vi "VIH HelpGen - Write HTML File - VI - VI Description.vi"(4 "InstanceRef":string, 6 "Description Params":cluster{"DscrMode":T3, "Description":string}, 7 "Save params":T1, 8 "error in":errorcluster, 9 "Original VI Info":cluster{"VI Name":string, "Conpane Image":T2}, 10 "HTML in":string, 11 "VI Reference":refnum<vi>) -> (0 "error out":errorcluster, 2 "HTML out":string, 3 "dup VI Reference":refnum<vi>)   [LabVIEW 2014]
doc: "::: VI Helpeks :::\nCopyright (c) 2000-2026 Konstantin Shifershteyn. All rights reserved."
uses:
  VIH HelpGen Typedef - Enum - Description Mode.ctl
  <vilib>/picture/picture.llb/imagedata.ctl
panel:
  out "ALL FOUND":bool
  # "VI Helpeks\nCopyright (c) 2012-2026 Konstantin Shifershteyn"
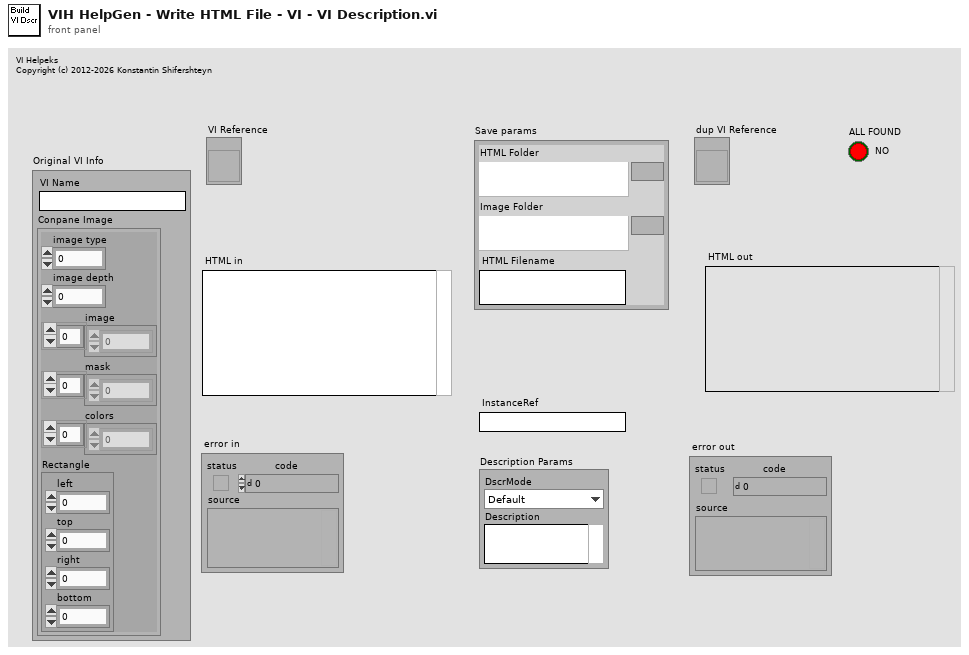
[diagram p1: front panel]
types:
  T1 = cluster{"HTML Folder":path, "Image Folder":path, "HTML Filename":string}
  T2 = typedef "imagedata.ctl" = cluster{"image type":i32, "image depth":i32, "image":u8[], "mask":u8[], "colors":u32[], "Rectangle":cluster{"left":i16, "top":i16, "right":i16, "bottom":i16}}
  T3 = typedef "VIH HelpGen Typedef - Enum - Description Mode.ctl" = enum16{"Default", "Description", "Description1", "Description2", "Custom", "None"}
  T4 = typedef "VIH HelpGen Typedef - Control Terminal Attributes Cluster.ctl" = cluster{"Conpane Idx":i32, "Control":bool, "Wire Rule":enum16{"Invalid Wire Rule", "Required", "Recommended", "Optional", "Dynamic Dispatch"}}
  T5 = cluster{"Ctrl ID":string, "Conpane Idx":i32, "Bounds":cluster{"X0":i32, "Y0":i32, "X1":i32, "Y1":i32}}[]
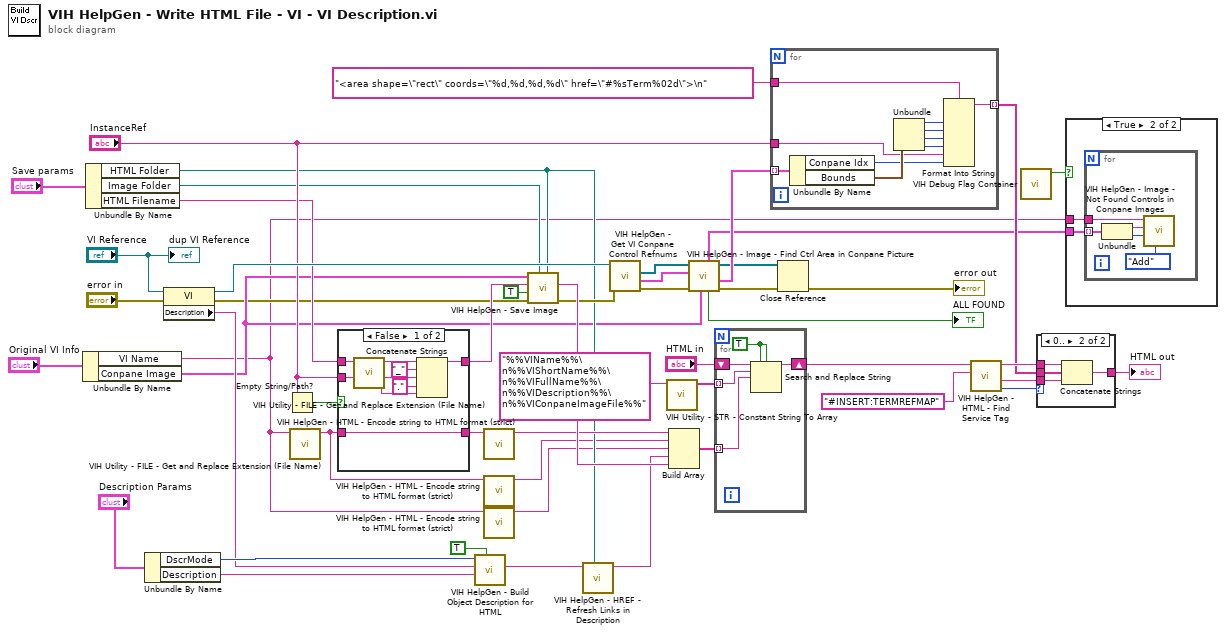
[diagram p0: block diagram]
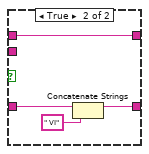
[diagram p3: hidden frame]
diagram:
  n1 = Unbundle By Name("Original VI Info") -> ("VI Name"=w4:string, "Conpane Image"=w6:T2)
  n2 = Unbundle By Name("Save params") -> ("HTML Folder"=w9:path, "Image Folder"=w8:path, "HTML Filename"=w7:string)
  n3 = Unbundle By Name("Description Params") -> ("DscrMode"=w27:T3, "Description"=w25:string)
  n4 = property class="VI"(reference="VI Reference", error in="error in") -> (reference out=w42:refnum<vi>, error out=w5:errorcluster, "Description"=w26:string)
  n5 = Empty String/Path?(string/path="InstanceRef") -> (empty?=w18:bool)
  n6 = call "VIH Utility - FILE - Get and Replace Extension (File Name).vi"("File name"=w4) -> ("File name out"=w3:string)  [unwired: 9 in, 1 out]
  n7 = case shown="False" w18 {
    tunnel: w3 -> [w59 w61]
    tunnel: [w59 w60] -> w14
    tunnel: [w58 w62] -> w11
    tunnel: w7 -> [w55 w62]
    tunnel: "InstanceRef" -> [w56 _]
    frame False {
      n8 = call "VIH Utility - FILE - Get and Replace Extension (File Name).vi"("File name"=w55) -> ("extension"=w53:string, "File name out"=w54:string)  [unwired: 9 in]
      n9 = Concatenate Strings(w54, "_" ("string"), w56, "." ("string"), w53) -> (w58:string)
    }
    frame True {
      n10 = Concatenate Strings(w61, " VI") -> (w60:string)
    }
  }
  n11 = call "VIH HelpGen - Build Object Description for HTML.vi"("Ena \"No Description\" message (F)"=TRUE ("Ena \"No Description\" message (F)"), "Custom Description"=w25, "Default Description"=w26, "DscrMode"=w27) -> ("Description HTML out"=w20:string)  [unwired: 6 in, 1 out]
  n12 = call "VIH HelpGen - HTML - Encode string to HTML format (strict).vi"("string"=w14) -> ("HTML string"=w13:string)  [unwired: 10 in]
  n13 = call "VIH HelpGen - HTML - Encode string to HTML format (strict).vi"("string"=w3) -> ("HTML string"=w2:string)  [unwired: 10 in]
  n14 = call "VIH HelpGen - HTML - Encode string to HTML format (strict).vi"("string"=w4) -> ("HTML string"=w1:string)  [unwired: 10 in]
  n15 = call "VIH HelpGen - Save Image.vi"("HTML Folder"=w9, "Image Folder"=w8, "error in"=w5, "Always overwrite (F)"=TRUE, "Image Filename"=w11, "image data"=w6) -> ("error out"=w43:errorcluster, "path for HTML"=w45:string)  [unwired: 3 in, 1 out]
  n16 = call "VIH HelpGen - HREF - Refresh Links in Description.vi"("HTML Folder"=w9, "Description in"=w20) -> ("Description out"=w19:string)  [unwired: 9 in]
  n17 = call "VIH HelpGen - Get VI Conpane Control Refnums.vi"("error in"=w43, "VI Reference"=w42) -> ("error out"=w41:errorcluster, "Ctrl Attributes"=w21:T4[], "Conpane Ctrl Refnums"=w23:refnum<vi>[])  [unwired: 6 in, 1 out]
  n18 = call "VIH Utility - STR - Constant String To Array.vi"("String in"="%%VIName%%\n%%VIShortName%%\n%%VIFullName%%\n%%VIDescription%%\n%%VIConpaneImageFile%%") -> ("Array out"=w49:string[])  [unwired: 10 in]
  n19 = Build Array(w13, w2, w1, w19, w45) -> (w48:string[])
  n20 = call "VIH HelpGen - Image - Find Ctrl Area in Conpane Picture.vi"("Conpane Image Data"=w6, "error in"=w41, "Ctrl Attributes"=w21, "Conpane Ctrl Refnums"=w23) -> ("error out"=w40:errorcluster, "Terminals Info"=w33:T5, "dup Conpane Ctrl Refnums"=w22:refnum<vi>[], "ALL FOUND"=→"ALL FOUND":bool, "Not Found"=w16:cluster{"Ctrl ID":string, "Conpane Idx":i32}[])  [unwired: 3 in]
  n21 = for {
    shift-right: [w67] -> w37
    shift-left: "HTML in" -> [w68]
    tunnel: w49 -> [w65] mode=indexing
    tunnel: w48 -> [w64] mode=indexing
    w66 = TRUE
    n22 = Search and Replace String(replace all?=w66, case sensitive?=w66, input string=w68, search string=w65, replace string=w64) -> (result string=w67:string)  [unwired: 3 in, 3 out]
  }
  n23 = for {
    tunnel: w33 -> [w78] mode=indexing
    tunnel: "<area shape=\"rect\" coords=\"%d,%d,%d,%d\" href=\"#%sTerm%02d\">\n" -> [w72]
    tunnel: [w71] -> w31 mode=indexing
    tunnel: "InstanceRef" -> [w69]
    n24 = Unbundle By Name(w78) -> ("Conpane Idx"=w70:i32, "Bounds"=w77:cluster{"X0":i32, "Y0":i32, "X1":i32, "Y1":i32})
    n25 = Unbundle(w77) -> ("X0"=w76:i32, "Y0"=w73:i32, "X1"=w74:i32, "Y1"=w75:i32)
    n26 = Format Into String(format string=w72, w76, w73, w74, w75, w69, w70) -> (resulting string=w71:string)  [unwired: 2 in, 1 out]
  }
  n27 = Close Reference(reference=w22, error in (no error)=w40) -> (error out=→"error out":errorcluster)
  n28 = call "VIH HelpGen - HTML - Find Service Tag.vi"("Tag name"="#INSERT:TERMREFMAP", "HTML in"=w37) -> ("Offset out"=w30:i32, "After"=w35:string, "Before"=w36:string)  [unwired: 6 in, 1 out]
  n29 = call "VIH Debug Flag Container.vi"() -> ("Debug Mode"=w15:bool)  [unwired: 11 in]
  n30 = case shown="0.." w30 {
    tunnel: w36 -> [w79 w83]
    tunnel: w35 -> [_ w82]
    tunnel: [w79 w81] -> w34
    tunnel: w31 -> [_ w80]
    frame ..-1 {
    }
    frame 0.. {
      n31 = Concatenate Strings(w83, w80, w82) -> (w81:string)
    }
  }
  "HTML out" <- w34
  n32 = case shown="True" w15 {
    tunnel: w16 -> [_ w85]
    tunnel: w4 -> [_ w84]
    frame False {
    }
    frame True {
      n33 = for {
        tunnel: w85 -> [w90] mode=indexing
        tunnel: w84 -> [w87]
        n34 = Unbundle(w90) -> ("Ctrl ID"=w88:string, "Conpane Idx"=w89:i32)
        n35 = call "VIH HelpGen - Image - Not Found Controls in Conpane Images.vi"("cmd"=enum16{"nop", "Init", "Add", "Show"}."Add", "Conpane Index"=w89, "Ctrl Name"=w88, "VI Name"=w87) -> ()  [unwired: 7 in, 1 out]
      }
    }
  }
  "dup VI Reference" <- "VI Reference"
